vi "CD Storage Library Unload.vi"(8 "error in (no error)":errorcluster, 11 "DMA Channel Testing in":refnum<class "FPGA Addon DMA Channel Unit Tests.lvclass">) -> (0 "error out":errorcluster, 3 "DMA Channel Testing out":refnum<class "FPGA Addon DMA Channel Unit Tests.lvclass">)   [LabVIEW 2020, in "FPGA Addon DMA Channel Unit Tests.lvclass"]
uses:
  FPGA Addon DMA Channel Unit Tests.lvclass
  FPGA Addon DMA Channel Unit Tests.lvclass/FPGA Addon DMA Channel Unit Tests.ctl
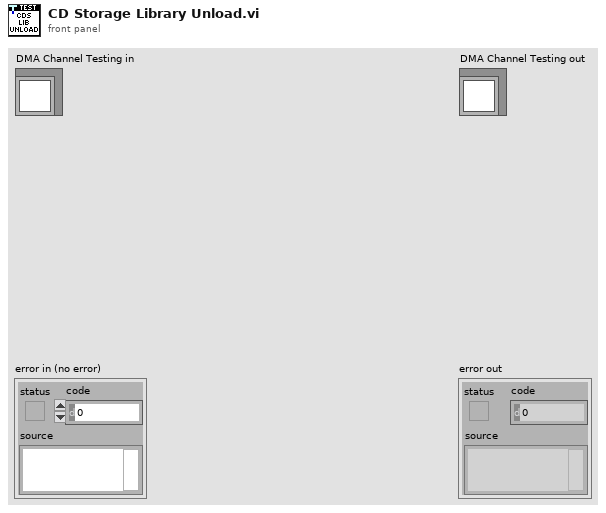
[diagram p1: front panel]
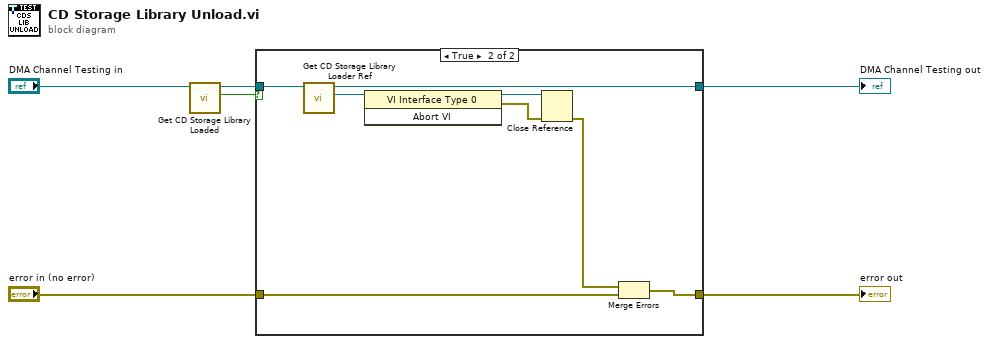
[diagram p0: block diagram]
diagram:
  n1 = call "Get CD Storage Library Loaded.vi"("DMA Channel Testing in"="DMA Channel Testing in") -> ("CDS Loaded"=w5:bool, "DMA Channel Testing out"=w4:refnum<class "FPGA Addon DMA Channel Unit Tests.lvclass">)  [unwired: 9 in]
  n2 = case shown="True" w5 {
    tunnel: w4 -> [w8 w16]
    tunnel: [w8 w14] -> w1
    tunnel: "error in (no error)" -> [w7 w13]
    tunnel: [w7 w11] -> w2
    frame False {
    }
    frame True {
      n3 = call "Get CD Storage Library Loader Ref.vi"("DMA Channel Testing in"=w16) -> ("CDS Loader Ref"=w15:refnum<vi>, "DMA Channel Testing out"=w14:refnum<class "FPGA Addon DMA Channel Unit Tests.lvclass">)  [unwired: 9 in]
      n4 = invoke class="VI Interface Type 0" method="Abort VI"(reference=w15) -> (reference out=w9:refnum<vi>, error out=w12:errorcluster)  [unwired: 2 in, 1 out]
      n5 = Close Reference(reference=w9, error in (no error)=w12) -> (error out=w10:errorcluster)
      n6 = Merge Errors(w10, w13) -> (w11:errorcluster)
    }
  }
  "error out" <- w2
  "DMA Channel Testing out" <- w1
